vi "Analog_Logger_Ex.vi"() -> ()   [LabVIEW 2026]
panel:
  in  "Intervalo (ms)":u32
  in  "file":path
  in  "Muestras":i32
  in  "VISA resource name":refnum<visa-resource-name>
  in  "Canal Read":u8
  out "Waveform Chart":i32(graph)
  out "error out":errorcluster
  # "Ejemplo: Analog Logger"
  # "Descripción: Registra en una gráfica y en un archivo las lecturas de un pin analógico del microcontrolador."
  # "Configuracion"
  # "Indicadores"
  # "Control"
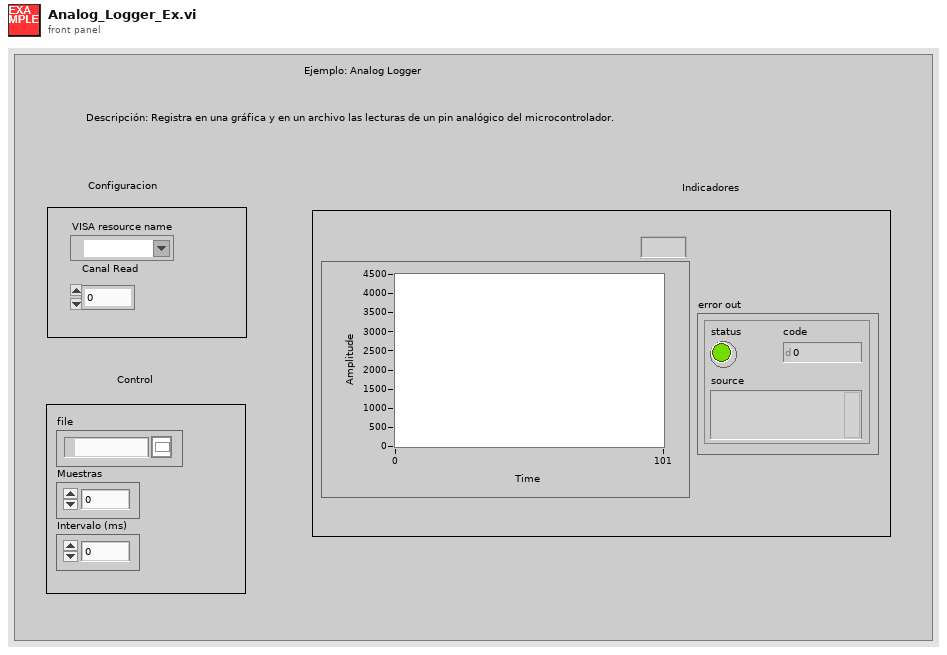
[diagram p1: front panel]
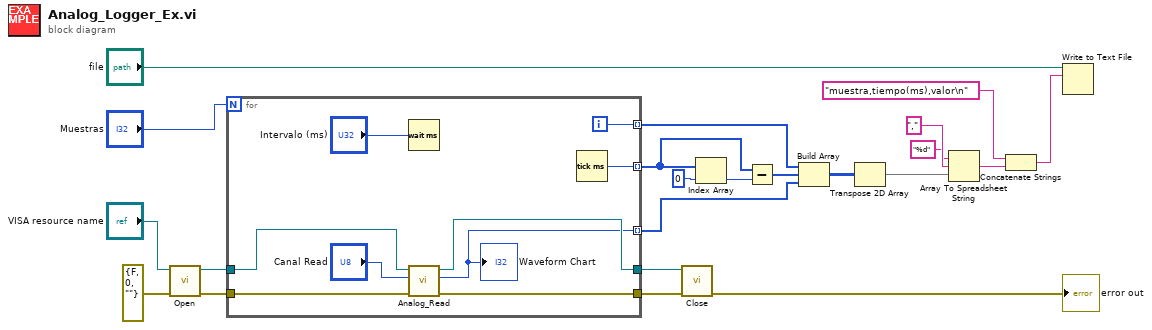
[diagram p0: block diagram]
diagram:
  n1 = call "Open.vi"("error in (no error)"=errorcluster {"status"=FALSE, "code"=0, "source"=""}, "VISA resource name"="VISA resource name") -> ("error out"=w22:errorcluster, "VISA resource name out"=w21:refnum<visa-resource-name>)  [unwired: 8 in]
  n2 = for {
    N: "Muestras" -> [_]
    tunnel: w22 -> [w30]
    tunnel: w21 -> [w29]
    tunnel: [w28] -> w16
    tunnel: [w27] -> w17
    tunnel: [w26] -> w2 mode=indexing
    tunnel: [w25] -> w9 mode=indexing
    tunnel: [w23] -> w4 mode=indexing
    i -> [w25]
    n3 = Wait (ms)(milliseconds to wait="Intervalo (ms)") -> ()  [unwired: 1 out]
    n4 = call "Analog_Read.vi"("error in (no error)"=w30, "Canal"="Canal Read", "VISA resource name"=w29) -> ("error out"=w28:errorcluster, "Out"=w26:i32, "VISA resource name out"=w27:refnum<visa-resource-name>)  [unwired: 6 in]
    "Waveform Chart" <- w26
    n5 = Tick Count (ms)() -> (millisecond timer value=w23:u32)
  }
  n6 = call "Close.vi"("error in (no error)"=w16, "VISA resource name"=w17) -> ("error out"=→"error out":errorcluster)  [unwired: 9 in]
  n7 = Index Array(array=w4, index=0) -> (element=w5:u32)
  n8 = Subtract(x=w4, y=w5) -> (x-y=w3:u32[])
  n9 = Build Array(w9, w3, w2) -> (w11:u32[][])
  n10 = Transpose 2D Array(2D array=w11) -> (transposed array=w10:u32[][])
  n11 = Array To Spreadsheet String(delimiter (Tab)=",", array=w10, 3:"%d" ("format string")) -> (spreadsheet string=w7:string)
  n12 = Concatenate Strings("muestra,tiempo(ms),valor\n", w7) -> (w1:string)
  n13 = Write to Text File(file (use dialog)="file", text=w1) -> ()  [unwired: 2 in, 3 out]
